vi "3_WF_Anomaly_Detection(Accuracy_Evaluation).vi"() -> ()   [LabVIEW 2020]
uses:
  <vilib>/Ngene/Deep Learning Toolkit/Toolkit/NN_Network/Controls/NN_Save_Before_Destroy_Options.ctl
  <vilib>/Ngene/Deep Learning Toolkit/Toolkit/NN_Data/subVIs/Dataset/NN_Variant_to_DVR/2D/NN_Data_Variant_to_DVR(2D_SGL).vi
  <vilib>/Ngene/Deep Learning Toolkit/Toolkit/NN_Network/subVIs/NN_Predict/NN_Predict(In1D_Out1D).vi
  <vilib>/Ngene/Deep Learning Toolkit/Toolkit/NN_Data/subVIs/Get_Data_Vals/2D/NN_Data_Get_ValByRef(2D_SGL).vi
  <vilib>/Ngene/Deep Learning Toolkit/Toolkit/Deep_Learning_Toolkit_by_Ngene.lvlib
  <vilib>/Analysis/NI_AALPro.lvlib
panel:
  out "Error Rate":sgl
  in  "Labels":string[](array[string])=["Normal", "Abnormal"]
  in  "Optimal Threshold":sgl=0.2
  out "Anomaly Score Distribution":T1(graph)=[{"X Values"=array[700 elements], "Histogram: h(x)"=[0, 0, 0, 0, 0, 0, 0, 0, 0, 0, 0, 0, 0, 0, 0, 0, 0, 0, 0, 0, 0, 0, 0, 0, 0, 0, 0, 0, 0, 0, 0, 0, 0, 0, 0, 1, 0, 1, 2, 2, 7, 7, 7, 4, 17, 6, 12, 11, 9, 10, 15, 15, 11, 18, 18, 18, 13, 13, 16, 11, 14, 20, 11, 9, 16, 11, 16, 10, 11, 9, 8, 15, 6, 8, 4, 10, 3, 4, 1, 6, 3, 6, 3, 10, 6, 5, 3, 1, 5, 2, 1, 2, 1, 4, 2, 2, 1, 1, 0, 1, 0, 0, 1, 0, 0, 0, 1, 1, 0, 0, 0, 0, 0, 0, 0, 0, 1, 0, 0, 0, 0, 0, 0, 1, 0, 0, 0, 0, 0, 0, 0, 0, 0, 0, 0, 0, 0, 0, 0, 0, 0, 0, 0, 0, 0, 0, 0, 0, 0, 0, 0, 0, 0, 0, 0, 0, 0, 0, 0, 0, 0, 0, 0, 0, 0, 0, 0, 0, 0, 0, 0, 0, 0, 0, 0, 0, 0, 0, 0, 0, 0, 0, 0, 0, 0, 0, 0, 0, 0, 0, 0, 0, 0, 0, 0, 0, 0, 0, 0, 0, 0, 0, 0, 0, 0, 0, 0, 0, 0, 0, 0, 0, 0, 0, 0, 0, 0, 0, 0, 0, 0, 0, 0, 0, 0, 0, 0, 0, 0, 0, 0, 0, 0, 0, 0, 0, 0, 0, 0, 0, 0, 0, 0, 0, 0, 0, 0, 0, 0, 0, 0, 0, 0, 0, 0, 0, 0, 0, 0, 0, 0, 0, 0, 0, 0, 0, 0, 0, 0, 0, 0, 0, 0, 0, 0, 0, 0, 0, 0, 0, 0, 0, 0, 0, 0, 0, 0, 0, 0, 0, 0, 0, 0, 0, 0, 0, 0, 0, 0, 0, 0, 0, 0, 0, 0, 0, 0, 0, 0, 0, 0, 0, 0, 0, 0, 0, 0, 0, 0, 0, 0, 0, 0, 0, 0, 0, 0, 0, 0, 0, 0, 0, 0, 0, 0, 0, 0, 0, 0, 0, 0, 0, 0, 0, 0, 0, 0, 0, 0, 0, 0, 0, 0, 0, 0, 0, 0, 0, 0, 0, 0, 0, 0, 0, 0, 0, 0, 0, 0, 0, 0, 0, 0, 0, 0, 0, 0, 0, 0, 0, 0, 0, 0, 0, 0, 0, 0, 0, 0, 0, 0, 0, 0, 0, 0, 0, 0, 0, 0, 0, 0, 0, 0, 0, 0, 0, 0, 0, 0, 0, 0, 0, 0, 0, 0, 0, 0, 0, 0, 0, 0, 0, 0, 0, 0, 0, 0, 0, 0, 0, 0, 0, 0, 0, 0, 0, 0, 0, 0, 0, 0, 0, 0, 0, 0, 0, 0, 0, 0, 0, 0, 0, 0, 0, 0, 0, 0, 0, 0, 0, 0, 0, 0, 0, 0, 0, 0, 0, 0, 0, 0, 0, 0, 0, 0, 0, 0, 0, 0, 0, 0, 0, 0, 0, 0, 0, 0, 0, 0, 0, 0, 0, 0, 0, 0, 0, 0, 0, 0, 0, 0, 0, 0, 0, 0, 0, 0, 0, 0, 0, 0, 0, 0, 0, 0, 0, 0, 0, 0, 0, 0, 0, 0, 0, 0, 0, 0, 0, 0, 0, 0, 0, 0, 0, 0, 0, 0, 0, 0, 0, 0, 0, 0, 0, 0, 0, 0, 0, 0, 0, 0, 0, 0, 0, 0, 0, 0, 0, 0, 0, 0, 0, 0, 0, 0, 0, 0, 0, 0, 0, 0, 0, 0, 0, 0, 0, 0, 0, 0, 0, 0, 0, 0, 0, 0, 0, 0, 0, 0, 0, 0, 0, 0, 0, 0, 0, 0, 0, 0, 0, 0, 0, 0, 0, 0, 0, 0, 0, 0, 0, 0, 0, 0, 0, 0, 0, 0, 0, 0, 0, 0, 0, 0, 0, 0, 0, 0, 0, 0, 0, 0, 0, 0, 0, 0, 0, 0, 0, 0, 0, 0, 0, 0, 0, 0, 0, 0, 0, 0, 0, 0, 0, 0, 0, 0, 0, 0, 0, 0, 0, 0, 0, 0, 0, 0, 0, 0, 0, 0, 0, 0, 0, 0, 0, 0, 0, 0, 0, 0, 0, 0, 0, 0, 0, 0, 0, 0, 0, 0, 0, 0, 0, 0, 0, 0, 0, 0, 0, 0, 0]}, {"X Values"=array[700 elements], "Histogram: h(x)"=[0, 0, 0, 0, 0, 0, 0, 0, 0, 0, 0, 0, 0, 0, 0, 0, 0, 0, 0, 0, 0, 0, 0, 0, 0, 0, 0, 0, 0, 0, 0, 0, 0, 0, 0, 0, 0, 0, 0, 0, 0, 0, 0, 0, 0, 0, 0, 0, 0, 0, 0, 0, 0, 0, 0, 0, 0, 0, 0, 0, 0, 0, 0, 0, 0, 0, 0, 0, 0, 0, 0, 0, 0, 0, 0, 0, 0, 0, 0, 0, 0, 0, 0, 0, 0, 0, 0, 0, 0, 0, 0, 0, 0, 0, 0, 0, 0, 0, 0, 0, 0, 0, 0, 0, 0, 0, 0, 0, 0, 0, 0, 0, 0, 0, 0, 0, 0, 0, 0, 0, 0, 0, 0, 0, 0, 0, 0, 0, 0, 0, 0, 0, 0, 0, 0, 0, 0, 0, 0, 0, 0, 0, 0, 0, 0, 0, 0, 0, 0, 0, 0, 0, 0, 0, 0, 0, 0, 0, 0, 0, 0, 0, 0, 0, 0, 0, 0, 0, 0, 1, 0, 0, 0, 0, 0, 2, 0, 0, 0, 0, 0, 0, 0, 0, 1, 1, 2, 1, 2, 0, 2, 0, 1, 0, 0, 0, 1, 1, 1, 1, 2, 3, 2, 0, 1, 0, 2, 3, 1, 2, 0, 4, 4, 1, 0, 1, 1, 0, 0, 0, 1, 0, 4, 3, 2, 5, 2, 2, 1, 1, 2, 1, 4, 3, 2, 1, 2, 5, 0, 4, 1, 1, 3, 2, 2, 2, 1, 2, 6, 2, 1, 0, 0, 2, 1, 3, 2, 3, 6, 1, 4, 5, 0, 1, 1, 4, 3, 2, 5, 2, 2, 0, 1, 0, 2, 0, 2, 4, 0, 2, 0, 2, 0, 4, 1, 0, 1, 1, 0, 1, 1, 3, 3, 1, 0, 0, 3, 1, 1, 0, 1, 1, 1, 4, 2, 2, 3, 0, 1, 1, 3, 1, 1, 0, 0, 0, 2, 0, 1, 3, 1, 0, 1, 1, 1, 0, 1, 0, 1, 1, 0, 0, 0, 0, 1, 2, 1, 0, 1, 0, 0, 0, 0, 0, 0, 0, 3, 2, 0, 0, 0, 1, 0, 0, 0, 2, 0, 0, 1, 0, 1, 2, 2, 4, 2, 1, 2, 3, 1, 1, 3, 0, 1, 3, 1, 2, 0, 1, 0, 1, 0, 2, 1, 1, 1, 2, 1, 0, 2, 0, 1, 1, 2, 4, 4, 2, 2, 0, 1, 2, 1, 1, 1, 1, 1, 1, 1, 1, 2, 1, 1, 1, 1, 5, 3, 1, 1, 1, 4, 2, 3, 1, 0, 0, 1, 0, 0, 0, 1, 5, 2, 1, 2, 1, 1, 3, 0, 3, 2, 2, 0, 1, 1, 2, 1, 0, 2, 1, 2, 0, 1, 0, 1, 2, 0, 1, 0, 0, 2, 0, 0, 0, 2, 1, 2, 1, 2, 1, 1, 1, 1, 0, 1, 1, 0, 1, 1, 0, 1, 1, 0, 0, 0, 0, 0, 1, 0, 0, 0, 1, 0, 0, 0, 0, 0, 0, 0, 0, 0, 0, 0, 1, 0, 0, 0, 0, 0, 0, 0, 0, 0, 1, 0, 0, 0, 0, 0, 0, 0, 0, 0, 0, 0, 0, 0, 0, 0, 0, 0, 0, 0, 0, 0, 0, 0, 0, 1, 0, 0, 0, 0, 0, 0, 0, 0, 0, 0, 0, 0, 0, 0, 0, 0, 0, 0, 0, 0, 0, 0, 0, 0, 0, 0, 0, 0, 0, 0, 1, 1, 0, 0, 0, 0, 0, 1, 1, 1, 0, 0, 0, 0, 0, 0, 1, 0, 0, 3, 0, 1, 0, 0, 0, 0, 2, 2, 0, 4, 0, 3, 3, 1, 0, 1, 4, 4, 1, 3, 1, 0, 2, 1, 2, 1, 3, 1, 1, 0, 1, 0, 5, 2, 4, 4, 2, 1, 1, 0, 1, 1, 2, 1, 2, 3, 2, 1, 1, 1, 3, 0, 0, 1, 4, 1, 0, 0, 2, 0, 0, 2, 0, 0, 0, 0, 0, 0, 1, 0, 0, 1, 0, 0, 0, 0, 0, 0, 0, 0, 0, 0, 0, 0, 0, 0, 0, 0, 0, 0, 0, 0, 0, 0, 0, 0, 0, 0, 0, 0, 0, 0, 0, 0, 0, 0, 0, 0, 0, 0, 0, 0, 0]}]
  in  "Test (Normal Samples) Dataset Folder path":path=path "D:/working/Anomaly Detection/Test/Normal"
  out "Confusion Matrix (Table)":string[][](table)=[["500", "0", "1.0000"], ["0", "500", "1.0000"], ["1.0000", "1.0000", ""]]
  in  "Test (Abnormal Samples) Dataset Folder path":path=path "D:/working/Anomaly Detection/Test/Abnormal"
  in  "Weights File Path":path=path "D:/Ngene/GitHub/deepltk_examples/2_Waveform_Processing/24_Waveform_Anomaly_Detection/working/Anomaly_Detection/Anomaly_Detection_weights_25_06_11__13_26_24.bin"
  in  "CFG file path":path=path "D:/Ngene/GitHub/deepltk_examples/2_Waveform_Processing/24_Waveform_Anomaly_Detection/working/Anomaly_Detection/Anomaly_Detection_net_cfg_25_06_11__13_26_24.cfg"
  # "Overview: This VI is designed to calculate the optimal anomaly threshold on the generated synthetic dataset.\nRequirements: Deep Learning Toolkit for LabVIEW - https://www.ngene.co/deep-learning-toolkit-for-labview\nInstructions:\n1. Provide \"Network Configuration File Path\" and \"Weight File Path\" generated from \"1_WF_Anomaly_Detection(Training).vi\".\n2. Provide Train and Test dataset paths.\n3. Run the VI.\n4.Observe the Range of optimal threshold values.\n5. Choose a value from the range of optimal threshold calculated after the VI stops, and use it as a anomaly detetcion threshold in \"3_WF_Anomaly_Detection(Threshold_Evaluation).vi\" \n6. Open \"3_WF_Anomaly_Detection(Inference).vi\"  to deploy the trained network for inference on manually generated samples."
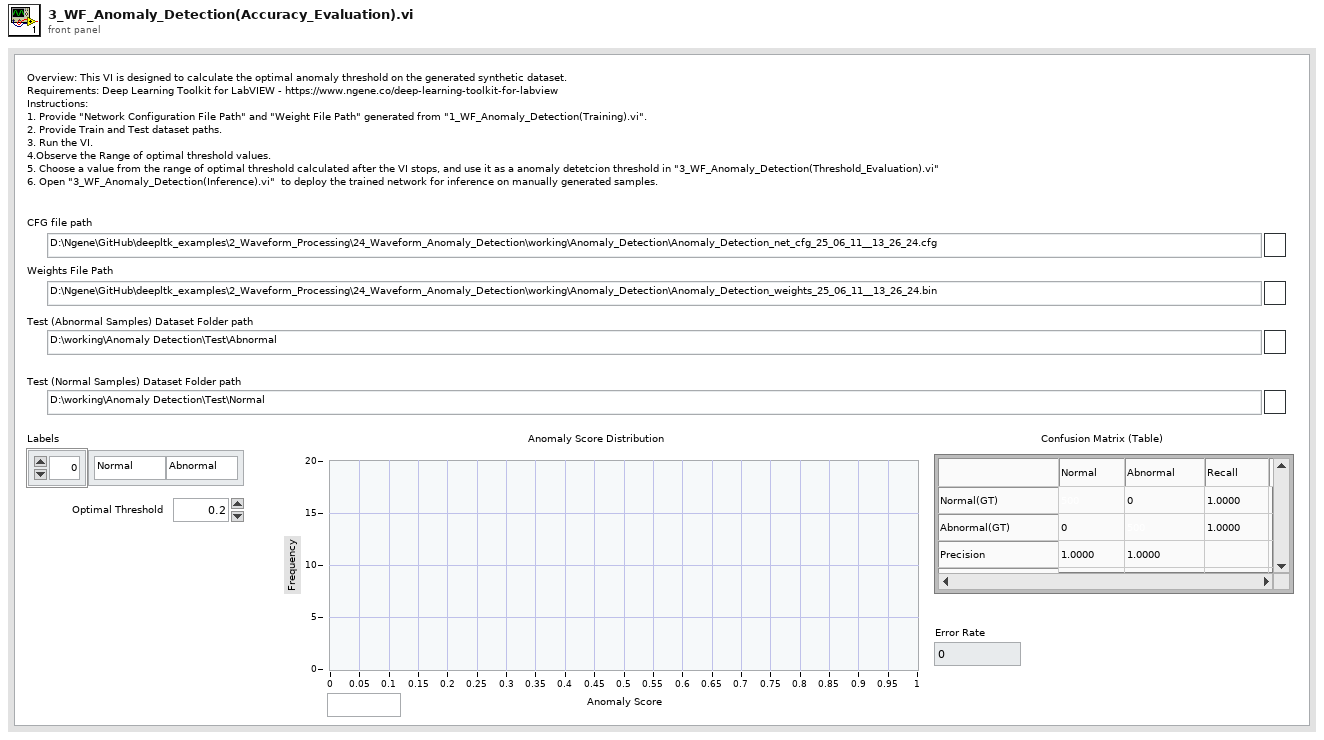
[diagram p1: front panel]
types:
  T1 = cluster{"X Values":dbl[], "Histogram: h(x)":i32[]}[]
  T2 = typedef "Deep_Learning_Toolkit_by_Ngene.lvlib/NN_Save_Before_Destroy_Options.ctl" = cluster{"CFG?":bool, "Weights?":bool, "Render?":bool}
  T3 = typedef "Deep_Learning_Toolkit_by_Ngene.lvlib/NN_Config_Params.ctl" = cluster{"Name":string, "mBatch":i32, "NN_Train_Params":T4, "LR_Decay_Policy":T7, "Labels":string[], "Loss":T9, "Max_WS_Size(B)":i64, "DryRun?":bool}
  T4 = typedef "Deep_Learning_Toolkit_by_Ngene.lvlib/NN_Train_Params.ctl" = cluster{"Optimizer":T5, "Beta_1":sgl, "Beta_2":sgl, "Weight Decay(L1)":sgl, "Weight Decay(L2)":sgl, "Data_Sampling":T6}
  T5 = typedef "Deep_Learning_Toolkit_by_Ngene.lvlib/NN_Train_Optimizer.ctl" = enum16{"SGD", "Adam", "Adagrad", "Adadelta", "RMSProp", "Nesterov"}
  T6 = typedef "Deep_Learning_Toolkit_by_Ngene.lvlib/NN_Train_Data_Sampling.ctl" = enum16{"Random", "Sequential"}
  T7 = typedef "Deep_Learning_Toolkit_by_Ngene.lvlib/NN_LR_Policy_Cfg.ctl" = cluster{"Policy_Type":T8, "LR0":dbl, "k":sgl, "WarmUp_Policy":enum16{"Step", "Ramp"}, "WarmUp_Iter":i32, "WarmUp_Ratio":sgl}
  T8 = typedef "Deep_Learning_Toolkit_by_Ngene.lvlib/NN_LR_Policy_Type.ctl" = enum16{"Manual", "Step", "Exp", "1/t"}
  T9 = typedef "Deep_Learning_Toolkit_by_Ngene.lvlib/NN_Loss_Config_Params.ctl" = cluster{"Loss_Type":T10, "Loss_Conf_Params":variant}
  T10 = typedef "Deep_Learning_Toolkit_by_Ngene.lvlib/NN_Loss_Type.ctl" = enum16{"None", "MSE", "CrossEntropy", "YOLO_v2", "YOLO_v4"}
  T11 = typedef "Deep_Learning_Toolkit_by_Ngene.lvlib/NN_Layer_Config_Params.ctl" = cluster{"Layer_Type":T12, "Layer_Conf_Params":variant, "Input Layers":string[]}
  T12 = typedef "Deep_Learning_Toolkit_by_Ngene.lvlib/NN_Layer_Type.ctl" = enum16{"Input1D", "Input3D", "Conv1D", "Conv2D", "Conv2D_Adv", "MaxPool", "AvgPool", "UpSample", "DropOut3D", "ShortCut", "Concat", "SoftMax3D", "FC", "DropOut", "Softmax", "Flatten", "YOLO_v2", "YOLO_v4", "Activation", "BatchNormalization", "LayerNormalization", "Scale", "Unsupported"}
  T13 = typedef "Deep_Learning_Toolkit_by_Ngene.lvlib/NN.ctl" = cluster{"Name":string, "No of Layers":i32, "mBatch":i32, "Layers":T14[], "Dimty":T15, "Dims_In":T16, "Dims_Out":T16, "Working_Dir":path, "Train?":bool, "Train_Params":T4, "LR_Update_Policy":T7, "Session Data":T17, "Ground_truth":T18, "NNg_hdls":T19, "NN_Device":T20, "GPU Id":i32, "Labels":string[], "Loss_Type":T10, "Loss_Cfg_Prms":variant, "NNG_WS":T21, "DryRun?":bool}
  T14 = typedef "Deep_Learning_Toolkit_by_Ngene.lvlib/NN_Layer_ref.ctl" = refnum<file>
  T15 = typedef "Deep_Learning_Toolkit_by_Ngene.lvlib/NN_In_Out_Dim-ty.ctl" = enum8{"In1D_Out1D", "In3D_Out1D", "In3D_Out3D", "In3D_OutBBox"}
  T16 = typedef "Deep_Learning_Toolkit_by_Ngene.lvlib/NN_Dims(C,H,W).ctl" = cluster{"C":i32, "H":i32, "W":i32}
  T17 = typedef "Deep_Learning_Toolkit_by_Ngene.lvlib/NN_Train_Session_Data.ctl" = cluster{"Epochs":sgl, "Tot_Iter":i32, "LR":sgl, "LR_iter":i32}
  T18 = typedef "Deep_Learning_Toolkit_by_Ngene.lvlib/NN_Ground_truth.ctl" = cluster{"Y":variant}
  T19 = typedef "Deep_Learning_Toolkit_by_Ngene.lvlib/nng_cuda_handles.ctl" = cluster{"cudnn":u64, "cublas":u64, "stream":u64, "curand":u64}
  T20 = typedef "Deep_Learning_Toolkit_by_Ngene.lvlib/NN_Device.ctl" = enum16{"CPU", "GPU"}
  T21 = typedef "Deep_Learning_Toolkit_by_Ngene.lvlib/NNG_WS.ctl" = cluster{"NNG_WS_Mem":T22, "Max_WS_Size":i64}
  T22 = typedef "Deep_Learning_Toolkit_by_Ngene.lvlib/NNg_WS_Mem_DVR.ctl" = refnum<data-value>
  T23 = typedef "Deep_Learning_Toolkit_by_Ngene.lvlib/NN_DataSet(In1D_Out1D).ctl" = cluster{"Inputs Ref.":variant, "Outputs Ref.":T24, "Dims_In":i32, "Dataset_Size":i32, "Dims_Out":i32, "Labels":string[], "File Paths":path[], "Custom_Data":variant}
  T24 = typedef "Deep_Learning_Toolkit_by_Ngene.lvlib/NN_Data_ref(2D_SGL).ctl" = refnum<data-value>
  T25 = cluster{"X Values":dbl[], "Histogram: h(x)":i32[]}
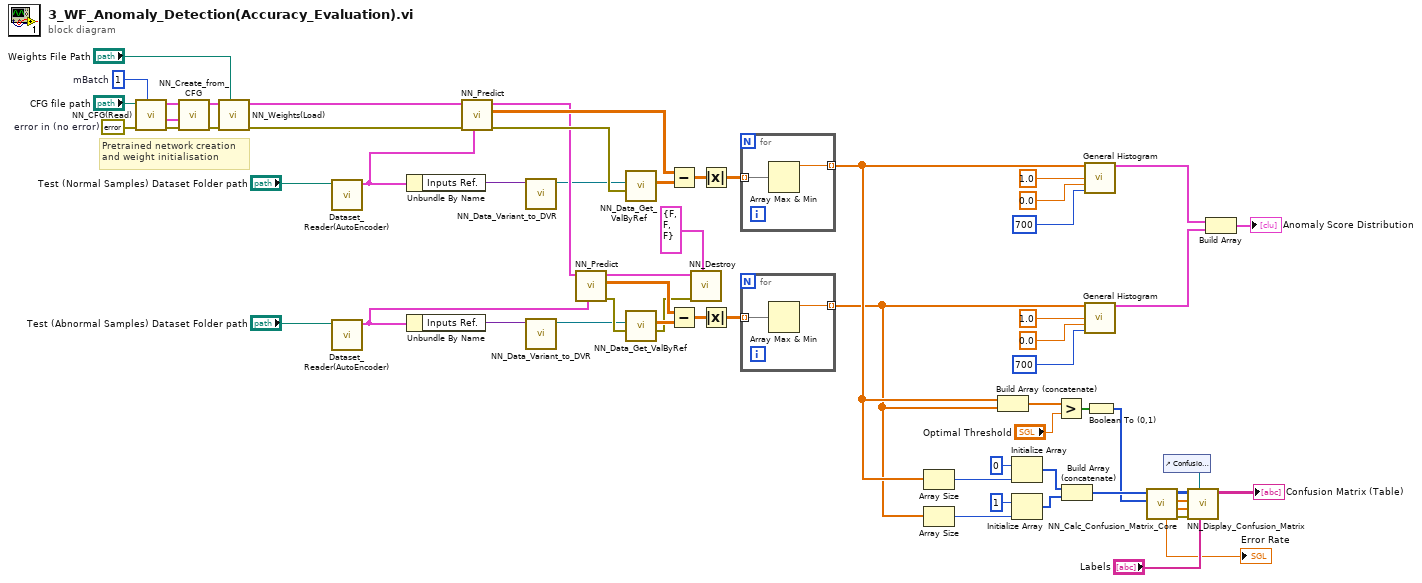
[diagram p0: block diagram]
diagram:
  w57 = 1  # mBatch
  w62 = errorcluster {"status"=FALSE, "code"=0, "source"=""}  # error in (no error)
  # "Pretrained network creation\nand weight initialisation"
  n1 = call <vilib>:"NN_CFG(Read).vi"("mBatch"=w57, "error in (no error)"=w62, "CFG file path"="CFG file path") -> ("error out"=w60:errorcluster, "Net_Cfg"=w61:T3, "Layer_Cfg"=w59:T11[])  [unwired: 6 in]
  n2 = call <vilib>:"NN_Create_from_CFG.vi"("error in (no error)"=w60, "Net_Cfg"=w61, "Layer_Cfg"=w59) -> ("error out"=w63:errorcluster, "NN out"=w58:T13)  [unwired: 7 in]
  n3 = call <vilib>:"NN_Weights(Load).vi"("Weight File Path"="Weights File Path", "error in (no error)"=w63, "NN in"=w58) -> ("error out"=w46:errorcluster, "NN out"=w47:T13)  [unwired: 7 in]
  n4 = call "Dataset_Reader(AutoEncoder).vi"("Train dataset path"="Test (Normal Samples) Dataset Folder path") -> ("Dataset"=w37:T23)  [unwired: 9 in, 1 out]
  n5 = call "Dataset_Reader(AutoEncoder).vi"("Train dataset path"="Test (Abnormal Samples) Dataset Folder path") -> ("Dataset"=w40:T23)  [unwired: 9 in, 1 out]
  n6 = Unbundle By Name(w37) -> ("Inputs Ref."=w44:variant)
  n7 = Unbundle By Name(w40) -> ("Inputs Ref."=w39:variant)
  n8 = call-poly <vilib>:"NN_Predict.vi"("Dataset"=w37, "error in (no error)"=w46, "NN in"=w47) -> ("error out"=w54:errorcluster, "Predictions"=w43:sgl[][], "NN out"=w41:T13)  [unwired: 6 in]
  n9 = call-poly <vilib>:"NN_Data_Variant_to_DVR.vi"("Inputs Ref."=w44) -> ("DVR(2D_SGL)"=w5:T24)  [unwired: 9 in, 1 out]
  n10 = call-poly <vilib>:"NN_Data_Variant_to_DVR.vi"("Inputs Ref."=w39) -> ("DVR(2D_SGL)"=w4:T24)  [unwired: 9 in, 1 out]
  n11 = call-poly <vilib>:"NN_Predict.vi"("Dataset"=w40, "NN in"=w41) -> ("error out"=w42:errorcluster, "Predictions"=w31:sgl[][], "NN out"=w3:T13)  [unwired: 7 in]
  n12 = call-poly <vilib>:"NN_Data_Get_ValByRef.vi"("error in (no error)"=w54, "DVR(2D_SGL)"=w5) -> ("Value(2D_SGL)"=w53:sgl[][])  [unwired: 6 in, 1 out]
  n13 = call-poly <vilib>:"NN_Data_Get_ValByRef.vi"("error in (no error)"=w42, "DVR(2D_SGL)"=w4) -> ("error out"=w2:errorcluster, "Value(2D_SGL)"=w32:sgl[][])  [unwired: 6 in]
  n14 = Subtract(x=w43, y=w53) -> (x-y=w52:sgl[][])
  n15 = Subtract(x=w31, y=w32) -> (x-y=w33:sgl[][])
  n16 = call <vilib>:"NN_Destroy.vi"("Save (T, T, T)"=T2 {"CFG?"=FALSE, "Weights?"=FALSE, "Render?"=FALSE}, "error in (no error)"=w2, "NN in"=w3) -> ()  [unwired: 7 in, 2 out]
  n17 = Absolute Value(x=w52) -> (abs(x)=w51:sgl[][])
  n18 = Absolute Value(x=w33) -> (abs(x)=w34:sgl[][])
  n19 = for {
    tunnel: w51 -> [w65] mode=indexing
    tunnel: [w64] -> w11 mode=indexing
    n20 = Array Max & Min(array=w65) -> (max value=w64:sgl)  [unwired: 3 out]
  }
  n21 = for {
    tunnel: w34 -> [w67] mode=indexing
    tunnel: [w66] -> w10 mode=indexing
    n22 = Array Max & Min(array=w67) -> (max value=w66:sgl)  [unwired: 3 out]
  }
  n23 = Array Size(array=w11) -> (size(s)=w20:i32)
  n24 = Array Size(array=w10) -> (size(s)=w15:i32)
  n25 = Build Array (concatenate)(w11, w10) -> (w12:sgl[])
  n26 = Initialize Array(0 ("element"), w20) -> (w18:i32[])
  n27 = Initialize Array(1 ("element"), w15) -> (w16:i32[])
  n28 = Greater?(x=w12, y="Optimal Threshold") -> (0:w9:bool[])
  n29 = Build Array (concatenate)(w18, w16) -> (w14:i32[])
  n30 = call <vilib>:"General Histogram.vi"("X"=w11, "max"=1.0, "min"=0.0, "# bins"=700) -> ("Histogram Graph"=w29:T25)  [unwired: 7 in, 4 out]
  n31 = call <vilib>:"General Histogram.vi"("X"=w10, "max"=1.0, "min"=0.0, "# bins"=700) -> ("Histogram Graph"=w28:T25)  [unwired: 7 in, 4 out]
  n32 = Boolean To (0,1)(Boolean=w9) -> (0, 1=w8:i16[])
  n33 = call <vilib>:"NN_Calc_Confusion_Matrix_Core.vi"("Predictions"=w8, "Ground_Truths"=w14) -> ("Error Out"=w23:errorcluster, "Recall"=w24:sgl[], "Precision"=w25:sgl[], "Confusion Matrix"=w26:i32[][], "Error Rate"=→"Error Rate":sgl)  [unwired: 5 in]
  n34 = control-ref of="Confusion Matrix (Table)"() -> (w22:refnum<vi>)
  n35 = call <vilib>:"NN_Display_Confusion_Matrix.vi"("Labels"="Labels", "Confusion Matrix (Table) ref"=w22, "error in (no error)"=w23, "Recall"=w24, "Precision"=w25, "Confusion Matrix"=w26) -> ("Confusion Matrix (Table)"=→"Confusion Matrix (Table)":string[][])  [unwired: 4 in, 1 out]
  n36 = Build Array(w29, w28) -> (→"Anomaly Score Distribution":T1)
